vi "process.vi"(8 "error in (no error)":errorcluster, 10 "Sync":refnum<notifier>, 11 "Session in":refnum<class "Session.lvclass">) -> (0 "error out":errorcluster, 3 "Session out":refnum<class "Session.lvclass">)   [LabVIEW 2013, in "MQTT Base.lvlib" / "Session.lvclass"]
uses:
  Session.lvclass
  Session.lvclass/Session.ctl
  DebuggingTerminal/Stream Direction -- enum.ctl
  Session Disconnection Reason -- enum.ctl
  <vilib>/LabVIEW Open Source Project/MQTT Control Packets/Control Packets/ControlPacket/ControlPacket.lvclass
  <vilib>/LabVIEW Open Source Project/MQTT Control Packets/Control Packets/MQTT_311/MQTTVersion.lvclass
  <vilib>/LabVIEW Open Source Project/Connection/Connection/Connection.lvclass
  DebuggingTerminal/DebuggingTerminal.lvclass
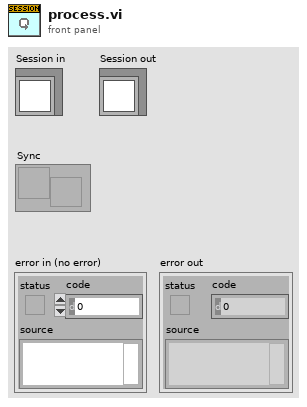
[diagram p1: front panel]
types:
  T1 = typedef "MQTT Base.lvlib/Session.lvclass/Session Disconnection Reason -- enum.ctl" = enum16{"Normal Stop", "Protocol Violation", "Disconnected by Peer"}
  T2 = typedef "MQTT Base.lvlib/DebuggingTerminal.lvclass/Stream Direction -- enum.ctl" = enum16{"Incoming", "Outgoing"}
  T3 = typedef "MQTT Base.lvlib/MQTT_Base.lvclass/Response -- cluster.ctl" = cluster{"Packet":refnum<class "ControlPacket.lvclass">, "Protocol Error":errorcluster, "disconnect session":bool, "[ACK]":refnum<notifier>[]}
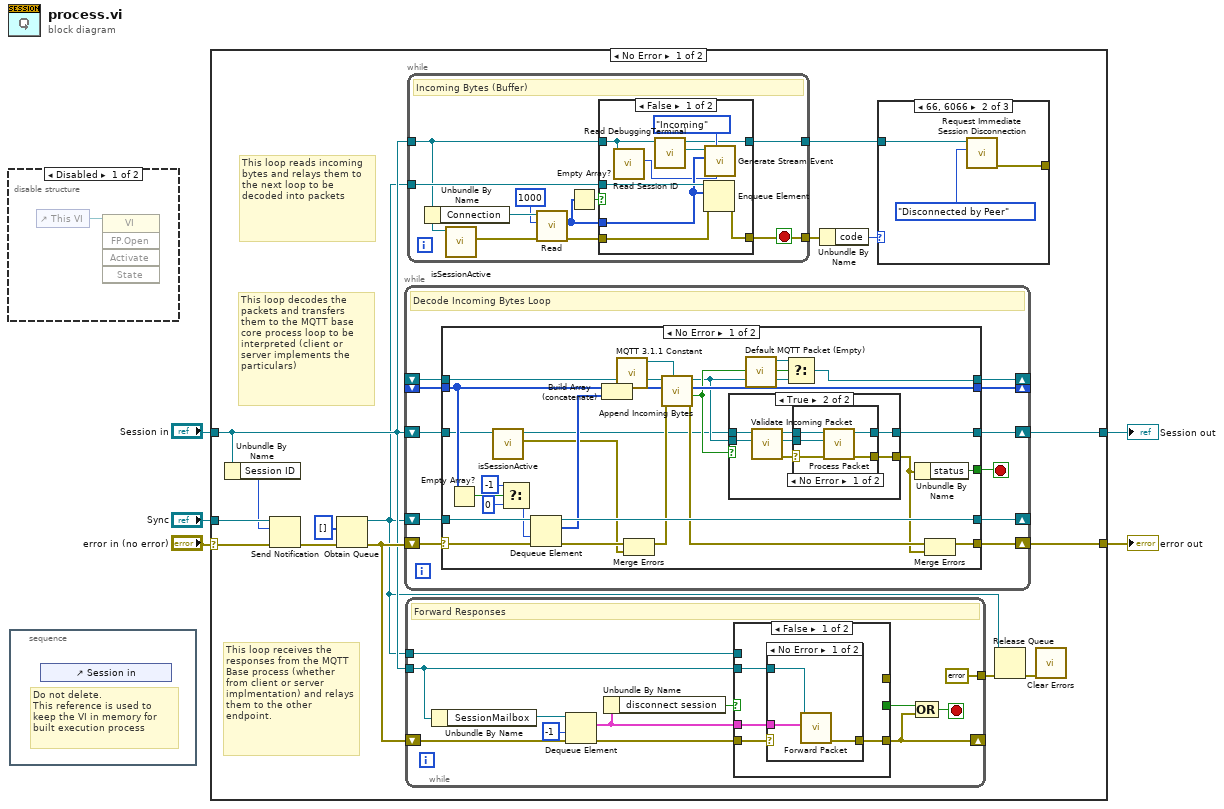
[diagram p0: block diagram]
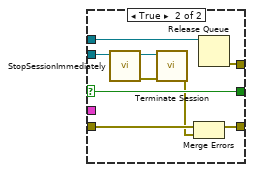
[diagram p4: hidden frame]
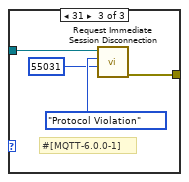
[diagram p6: hidden frame]
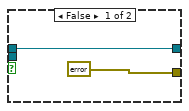
[diagram p8: hidden frame]
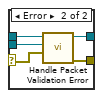
[diagram p9: hidden frame]
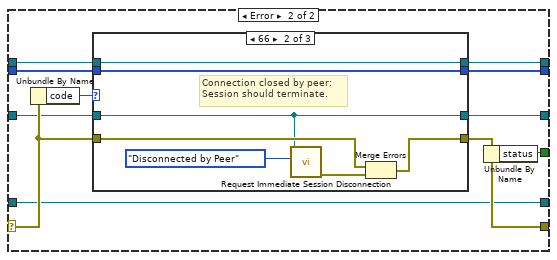
[diagram p10: hidden frame]
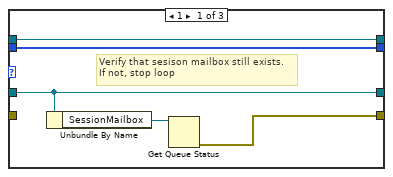
[diagram p11: hidden frame]
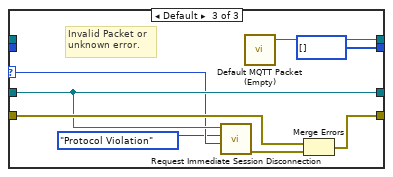
[diagram p12: hidden frame]
diagram:
  n1 = disable-structure shown="Disabled" {
    frame Disabled {
      n2 = control-ref of="This VI"() -> (w6:refnum<vi>)
      n3 = invoke class="VI" method="FP.Open"(reference=w6) -> ()  [unwired: 4 in, 5 out]
    }
    frame Enabled {
    }
  }
  n4 = stacked-sequence {
    frame #0 {
      # "Do not delete.\nThis reference is used to keep the VI in memory for built execution process"
      n5 = control-ref of="Session in"() -> ()  [unwired: 1 out]
    }
  }
  n6 = case shown="No Error" "error in (no error)" {
    selector: "error in (no error)" -> [w20 w168]
    tunnel: [w13 w168] -> w1
    tunnel: [w15 w167] -> w3
    tunnel: "Session in" -> [w11 w167]
    tunnel: "Sync" -> [w21 _]
    frame No Error {
      # "This loop receives the responses from the MQTT Base process (whether from client or server implmentation) and relays them to the other endpoint."
      # "This loop decodes the packets and transfers them to the MQTT base core process loop to be interpreted (client or server implements the particulars)"
      # "This loop reads incoming bytes and relays them to the next loop to be decoded into packets"
      n7 = Unbundle By Name(w11) -> ("Session ID"=w12:i32)
      n8 = Send Notification(notification=w12, notifier=w21, error in (no error)=w20) -> (error out=w14:errorcluster)  [unwired: 1 out]
      n9 = Obtain Queue(element data type=u8[] [] ("Remaining Packets"), error in (no error)=w14) -> (queue out=w8:refnum<queue>, error out=w19:errorcluster)  [unwired: 3 in, 1 out]
      n10 = while {
        shift-right: [w87] -> _
        shift-left: _ -> [w86]
        shift-right: [w85] -> w13
        shift-left: w19 -> [w84]
        shift-right: [w88] -> _
        shift-left: _ -> [w89]
        shift-right: [w81] -> _
        shift-left: w8 -> [w82]
        shift-right: [w79] -> w15
        shift-left: w11 -> [w80]
        stop <- w83 stop-if-true
        # "Decode Incoming Bytes Loop"
        n11 = case shown="No Error" w84 {
          selector: w84 -> [w109 w144]
          tunnel: w89 -> [w116 w142]
          tunnel: [w101 w146] -> w88
          tunnel: [w114 w145] -> w87
          tunnel: w86 -> [w106 w136]
          tunnel: [w107 w141] -> w85
          tunnel: [w95 w140] -> w83
          tunnel: w82 -> [w113 w139]
          tunnel: [w112 w139] -> w81
          tunnel: w80 -> [w92 w138]
          tunnel: [w97 w137] -> w79
          frame No Error {
            # "No Error"
            n12 = Empty Array?(array=w106) -> (empty?=w105:bool)
            n13 = call "isSessionActive.vi"("Session in"=w92) -> ("error out"=w90:errorcluster, "Session out"=w91:refnum<class "Session.lvclass">)  [unwired: 9 in]
            n14 = Select(t=-1 ("timeout in ms (-1)"), s=w105, f=0) -> (s? t:f=w103:i32)
            n15 = Dequeue Element(queue=w113, timeout in ms (-1)=w103, error in (no error)=w109) -> (queue out=w112:refnum<queue>, element=w111:u8[], error out=w94:errorcluster)  [unwired: 1 out]
            n16 = Build Array (concatenate)(w106, w111) -> (w110:u8[])
            n17 = call <vilib>:"MQTT 3.1.1 Constant.vi"() -> ("MQTT 3.1.1"=w115:refnum<class "MQTTVersion.lvclass">)  [unwired: 11 in]
            n18 = Merge Errors(w94, w90) -> (w93:errorcluster)
            n19 = call <vilib>:"Append Incoming Bytes.vi"("MQTT Version (3.1.1)"=w115, "error in (no error)"=w93, "Incoming Packets"=w110, "Incomplete ControlPacket"=w116) -> ("error out"=w108:errorcluster, "Complete Packet"=w99:bool, "Remaining Packets"=w114:u8[], "ControlPacket"=w98:refnum<class "ControlPacket.lvclass">)  [unwired: 4 in]
            n20 = case shown="True" w99 {
              tunnel: [errorcluster {"status"=FALSE, "code"=0, "source"=""} ("error out") w119] -> w96
              tunnel: w98 -> [_ w125]
              tunnel: w91 -> [w117 w124]
              tunnel: [w117 w120] -> w97
              frame False {
                # "No Packet received"
              }
              frame True {
                # "Packet Received"
                n21 = call-dynamic "Validate Incoming Packet.vi"("ControlPacket"=w125, "Session in"=w124) -> ("error out"=w121:errorcluster, "ControlPacket out"=w122:refnum<class "ControlPacket.lvclass">, "Session out"=w123:refnum<class "Session.lvclass">)  [unwired: 7 in]
                n22 = case shown="No Error" w121 {
                  selector: w121 -> [w126 w133]
                  tunnel: [w127 w131] -> w120
                  tunnel: w123 -> [w130 w135]
                  tunnel: w122 -> [w129 w134]
                  tunnel: [w128 w132] -> w119
                  frame No Error {
                    n23 = call-dynamic "Process Packet.vi"("error in (no error)"=w126, "Incoming Packet"=w129, "Session in"=w130) -> ("error out"=w128:errorcluster, "Session out"=w127:refnum<class "Session.lvclass">)  [unwired: 7 in]
                  }
                  frame Error {
                    n24 = call "Handle Packet Validation Error.vi"("Packet Validation Error"=w133, "ControlPacket"=w134, "Session in"=w135) -> ("error out"=w132:errorcluster, "Session out"=w131:refnum<class "Session.lvclass">)  [unwired: 7 in]
                  }
                }
              }
            }
            n25 = call <vilib>:"Default MQTT Packet (Empty).vi"() -> ("No Packet"=w100:refnum<class "ControlPacket.lvclass">)  [unwired: 11 in]
            n26 = Select(t=w100, s=w99, f=w98) -> (s? t:f=w101:refnum<class "ControlPacket.lvclass">)
            n27 = Unbundle By Name(w96) -> ("status"=w95:bool)
            n28 = Merge Errors(w108, w96) -> (w107:errorcluster)
          }
          frame Error {
            # "Handle Error"
            n29 = Unbundle By Name(w144) -> ("code"=w143:i32)
            n30 = case shown="66" w143 {
              selector: w143 -> [_ _ w161]
              tunnel: [w150 w158 w164] -> w146
              tunnel: w144 -> [_ w156 w166]
              tunnel: [w147 w155 w165] -> w141
              tunnel: [w149 w157 u8[] [] ("Remaining Packets")] -> w145
              tunnel: w142 -> [w150 w158 _]
              tunnel: w138 -> [w148 w153 w162]
              tunnel: [w148 w153 w162] -> w137
              tunnel: w136 -> [w149 w157 _]
              frame 1 {
                # "Verify that sesison mailbox still exists.\nIf not, stop loop"
                n31 = Unbundle By Name(w148) -> ("SessionMailbox"=w151:refnum<queue>)
                n32 = Get Queue Status(queue=w151) -> (error out=w147:errorcluster)  [unwired: 2 in, 7 out]
              }
              frame 66 {
                # "Connection closed by peer:\nSession should terminate."
                n33 = call "Request Immediate Session Disconnection.vi"("Disconnection Reason"=Session_Disconnection_Reason_--_enum."Disconnected by Peer", "Session in"=w153) -> ("error out"=w154:errorcluster)  [unwired: 8 in, 1 out]
                n34 = Merge Errors(w156, w154) -> (w155:errorcluster)
              }
              frame Default {
                # "Invalid Packet or\nunknown error."
                n35 = call "Request Immediate Session Disconnection.vi"("Protocol Violation Error Code"=w161, "Disconnection Reason"=Session_Disconnection_Reason_--_enum."Protocol Violation", "Session in"=w162) -> ("error out"=w160:errorcluster)  [unwired: 7 in, 1 out]
                n36 = call <vilib>:"Default MQTT Packet (Empty).vi"() -> ("No Packet"=w164:refnum<class "ControlPacket.lvclass">)  [unwired: 11 in]
                n37 = Merge Errors(w166, w160) -> (w165:errorcluster)
              }
            }
            n38 = Unbundle By Name(w141) -> ("status"=w140:bool)
          }
        }
      }
      n39 = while {
        tunnel: w11 -> [w29]
        shift-right: [w26] -> _
        shift-left: w19 -> [w30]
        tunnel: w8 -> [w23]
        tunnel: [errorcluster {"status"=FALSE, "code"=0, "source"=""} ("error IO")] -> w9
        stop <- w25 stop-if-true
        # "Forward Responses"
        n40 = Unbundle By Name(w29) -> ("SessionMailbox"=w33:refnum<queue>)
        n41 = Dequeue Element(queue=w33, timeout in ms (-1)=-1, error in (no error)=w30) -> (element=w28:T3, error out=w31:errorcluster)  [unwired: 2 out]
        n42 = Unbundle By Name(w28) -> ("disconnect session"=w27:bool)
        n43 = case shown="False" w27 {
          selector: w27 -> [_ w50]
          tunnel: w31 -> [w37 w48]
          tunnel: [w36 w47] -> w26
          tunnel: w29 -> [w35 w49]
          tunnel: w28 -> [w34 _]
          tunnel: [_ w50] -> w24
          tunnel: w23 -> [_ w43]
          tunnel: [_ w42] -> _
          frame False {
            n44 = case shown="No Error" w37 {
              selector: w37 -> [_ w41]
              tunnel: w34 -> [w39 _]
              tunnel: [w38 w41] -> w36
              tunnel: w35 -> [w40 _]
              frame No Error {
                n45 = call-dynamic "Forward Packet.vi"("Response"=w39, "Session in"=w40) -> ("error out"=w38:errorcluster)  [unwired: 9 in]
              }
              frame Error {
              }
            }
          }
          frame True {
            n46 = call "StopSessionImmediately.vi"("Session in"=w49) -> ("error out"=w45:errorcluster, "Session out"=w46:refnum<class "Session.lvclass">)  [unwired: 9 in]
            n47 = call "Terminate Session.vi"("error in (no error)"=w45, "Session in"=w46) -> ("error out"=w44:errorcluster)  [unwired: 7 in, 2 out]
            n48 = Merge Errors(w48, w44) -> (w47:errorcluster)
            n49 = Release Queue(queue=w43) -> (error out=w42:errorcluster)  [unwired: 2 in, 2 out]
          }
        }
        n50 = Compound Arithmetic op=OR(w24, w26) -> (w25:bool)
      }
      n51 = while {
        tunnel: w11 -> [w62]
        tunnel: [w58] -> w17
        tunnel: [w61] -> w10
        tunnel: w8 -> [w67]
        stop <- w58 stop-if-true
        # "Incoming Bytes (Buffer)"
        n52 = Unbundle By Name(w62) -> ("Connection"=w66:refnum<class "Connection.lvclass">)
        n53 = call "isSessionActive.vi"("Session in"=w62) -> ("error out"=w64:errorcluster)  [unwired: 9 in, 1 out]
        n54 = call <vilib>:"Read.vi"("error in (no error)"=w64, "bytes to read (100)"=1000, "TCPConnection in"=w66) -> ("error out"=w63:errorcluster, "Bytes"=w60:u8[])  [unwired: 4 in, 3 out]
        n55 = Empty Array?(array=w60) -> (empty?=w59:bool)
        n56 = case shown="False" w59 {
          tunnel: w67 -> [w76 _]
          tunnel: [w75 w77] -> w58
          tunnel: w63 -> [w74 w77]
          tunnel: w62 -> [w69 w78]
          tunnel: [w71 w78] -> w61
          tunnel: w60 -> [w70 _]
          frame False {
            n57 = call "Read Session ID.vi"("Session in"=w69) -> ("Session ID"=w68:i32)  [unwired: 8 in, 2 out]
            n58 = call "Read DebuggingTerminal.vi"("Session in"=w69) -> ("DebuggingTerminal"=w73:refnum<class "DebuggingTerminal.lvclass">, "Session out"=w71:refnum<class "Session.lvclass">)  [unwired: 8 in, 1 out]
            n59 = Enqueue Element(queue=w76, element=w70, error in (no error)=w74) -> (error out=w75:errorcluster)  [unwired: 1 in, 2 out]
            n60 = call "Generate Stream Event.vi"("Session ID"=w68, "Direction"=Stream_Direction_--_enum."Incoming", "Bytes"=w70, "DebuggingTerminal in"=w73) -> ()  [unwired: 6 in, 2 out]
          }
          frame True {
          }
        }
      }
      n61 = Unbundle By Name(w17) -> ("code"=w18:i32)
      n62 = case shown="66, 6066" w18 {
        tunnel: w10 -> [_ w53 w57]
        tunnel: [_ w51 w55] -> _
        frame Default {
        }
        frame 66, 6066 {
          n63 = call "Request Immediate Session Disconnection.vi"("Disconnection Reason"=Session_Disconnection_Reason_--_enum."Disconnected by Peer", "Session in"=w53) -> ("error out"=w51:errorcluster)  [unwired: 8 in, 1 out]
        }
        frame 31 {
          # "#[MQTT-6.0.0-1]"
          n64 = call "Request Immediate Session Disconnection.vi"("Protocol Violation Error Code"=55031, "Disconnection Reason"=Session_Disconnection_Reason_--_enum."Protocol Violation", "Session in"=w57) -> ("error out"=w55:errorcluster)  [unwired: 7 in, 1 out]
        }
      }
      n65 = Release Queue(queue=w8, error in (no error)=w9) -> (error out=w7:errorcluster)  [unwired: 1 in, 2 out]
      n66 = call <vilib>:"Clear Errors.vi"("error in (no error)"=w7) -> ()  [unwired: 6 in, 1 out]
    }
    frame Error {
    }
  }
  "error out" <- w1
  "Session out" <- w3
